vi "Generate cRIO-9068 Bitfile Path.vi"() -> (0 "Bitfile Path":path)   [LabVIEW 2020, in "FPGA Addon Load And Parse Bitfile Unit Tests.lvclass"]
uses:
  FPGA Addon Load And Parse Bitfile Unit Tests.lvclass
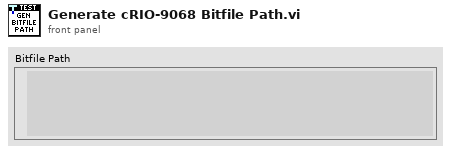
[diagram p1: front panel]
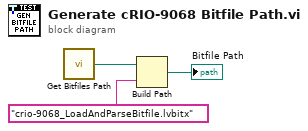
[diagram p0: block diagram]
diagram:
  n1 = call "Get Bitfiles Path.vi"() -> ("Bitfiles path"=w3:path)
  n2 = Build Path(base path=w3, name or relative path="crio-9068_LoadAndParseBitfile.lvbitx") -> (appended path=→"Bitfile Path":path)
